vi "Load.vi"(8 "error in (no error)":errorcluster, 11 "Tool in":refnum<class "ITool.lvclass">) -> (0 "error out":errorcluster, 2 "OpenTool":variant, 3 "Tool out":refnum<class "ITool.lvclass">)   [LabVIEW 2017, in "ITool.lvclass"]
uses:
  ITool.lvclass
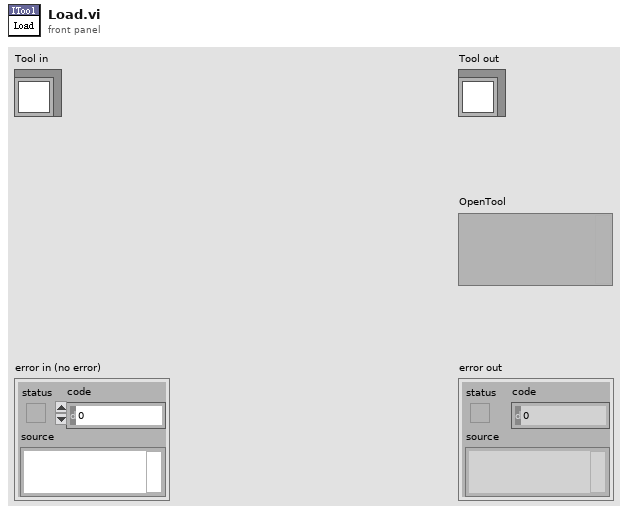
[diagram p1: front panel]
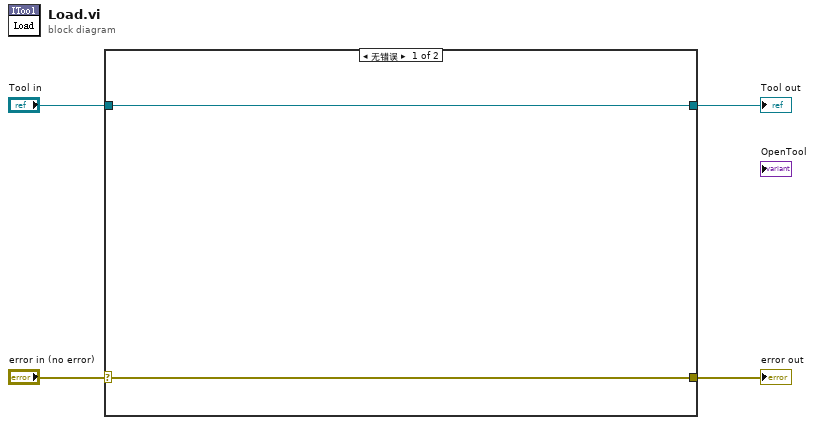
[diagram p0: block diagram]
diagram:
  n1 = case shown="无错误" "error in (no error)" {
    selector: "error in (no error)" -> [w5 w8]
    tunnel: [w5 w8] -> w1
    tunnel: [w6 w7] -> w3
    tunnel: "Tool in" -> [w6 w7]
    frame No Error {
    }
    frame Error {
    }
  }
  "Tool out" <- w3
  "error out" <- w1
